vi "1_10_Racing_Main.vi"() -> ()   [LabVIEW 2024]
uses:
  <vilib>/vision/Measure.llb/Edge New.ctl
  <vilib>/vision/Measure.llb/Edge Options.ctl
  <vilib>/vision/Measure.llb/Edge Polarity.ctl
  <vilib>/Instr/_visa.llb/VISA Set IO Buffer Mask.ctl
  <vilib>/Instr/_visa.llb/VISA Flush IO Buffer Mask.ctl
  <vilib>/Platform/TimedLoop/XDataNode/timing_clust.ctl
  <vilib>/Platform/TimedLoop/XDataNode/nitl_modes.ctl
  <vilib>/Platform/TimedLoop/XDataNode/wakeup.ctl
  <vilib>/Analysis/geometry.llb/Point in Polygon (Array).vi
  <vilib>/Instr/_visa.llb/VISA Configure Serial Port (Instr).vi
  <vilib>/Utility/file.llb/Write Delimited Spreadsheet (string).vi
  <vilib>/Platform/TimedLoop/XDataNode/XDataNode.xnode
  <vilib>/Analysis/NI_AAL_Geometry.lvlib
  <vilib>/ptbypt/NI_PtbyPt.lvlib
  <vilib>/Platform/TimedLoop/XDataNode/XDNodeRunTimeDep.lvlib
panel:
  out "curve":bool
  out "3":bool
  out "1":bool
  out "2":bool
  in  "Tab Control":T1(tab)=enum."oCam"
  in  "RP2040_Com.":refnum<visa-resource-name>="COM1"
  in  "LiDAR_Com.":refnum<visa-resource-name>="COM7"
  in  "HLV_EStop":bool
  in  "HLV_AorM":bool=TRUE
  out "Alive_PCU":u8(slide)=187 scale=0.0..254.0
  out "PCU_GEAR":u8
  in  "HLV_GEAR":u8(slide) scale=0.0..2.0
  in  "HLV_SPEED(mps)":i16(slide)=180 scale=0.0..1000.0
  out "PCU_MODE":u8=1
  out "PCU_SPEED (mps)":dbl=0.41000000000000003
  out "PCU_STEER":i16=-1108
  in  "pure_Y":dbl=0.93
  in  "L":dbl=0.288
  in  "LAD":dbl=0.93
  out "PCU_EStop":bool
  out "PCU_ENC":i32=1739477
  out "pure_CMD(Deg)":dbl=-17.928890679668594
  out "steer(pwm)":i16=-1115
  out "LiDAR E-STOP":bool
  in  "pure_gain":dbl=1.0
  in  "stanley_Y":dbl=0.67
  in  "stanley_gain":dbl=1.0
  in  "stanley_speed":dbl=36.0
  in  "pure_min":dbl=0.38
  in  "steer_mean_size":i8=1
  out "stanley_CMD(Deg)":dbl=-0.8745447541552979
  out "Output_Spd_CMD(pwm)":dbl=163.8
  out "Near Point":dbl=-0.56975
  in  "stanley_con":dbl=0.023
  out "steer(deg)":i16(knob)=-16 scale=-25.0..25.0
  out "하위제어기 통신 패킷":string
  out "TX Data Cnt (byte)":u32=13
  out "RX Data Cnt (byte)":u32=17
  out "string":string
  in  "voxelsize":dbl=0.05
  out "Loop Time":u32=100
  out "Loop Time 2":u32=97
  out "LiDAR_ROI":cluster{"Array 2":dbl[], "Array":dbl[]}[](graph)=[{"Array 2"=[-650.0, -250.0, -250.0, -650.0, -650.0], "Array"=[-500.0, -500.0, 1000.0, 1000.0, -500.0]}, {"Array 2"=[], "Array"=[]}, {"Array 2"=[-200.0, 200.0, 200.0, -200.0, -200.0], "Array"=[280.0, 280.0, 1000.0, 1000.0, 280.0]}, {"Array 2"=[], "Array"=[]}, {"Array 2"=[250.0, 650.0, 650.0, 250.0, 250.0], "Array"=[-500.0, -500.0, 1000.0, 1000.0, -500.0]}, {"Array 2"=[], "Array"=[]}, {"Array 2"=[-200.0, 200.0, 200.0, -200.0, -200.0], "Array"=[80.0, 80.0, 280.0, 280.0, 80.0]}, {"Array 2"=[], "Array"=[]}]
  in  "euclid":dbl=200.0 format="%#_13g"
  in  "max_cluster_size":dbl=500.0 format="%#_13g"
  out "f_dis(m)":dbl[](array[numeric])
  out "right_edge_location":cluster{"X":sgl, "Y":sgl}[](array[cluster])=[{"X"=620.9575, "Y"=283.14465}, {"X"=620.9575, "Y"=283.14465}]
  out "left_edge_location":cluster{"X":sgl, "Y":sgl}[](array[cluster])
  out "mid_edge_location":cluster{"X":sgl, "Y":sgl}[](array[cluster])=[{"X"=95.05083, "Y"=287.6531}, {"X"=114.194305, "Y"=282.5482}]
  out "target center":dbl=105.0
  out "mid_line_edge":i32=105
  out "right_roi_dead":bool
  out "left_roi_dead":bool=TRUE
  out "right_line_edge":i32=621
  out "left_line_edge":i32
  out "mid_roi_dead":bool
  out "mid_far_edge":i32=634
  out "mid_near_edge":i32=539
  out "Image Out":T2(plugin-control)
  out "L_color":string="None"
  out "R_color":string="None"
  out "Right Edge Information":T3[](array[typedef])=[{"Location (Pixel)"={"X"=620.9575, "Y"=283.14465}, "Location (Real-World)"={"X"=620.9575, "Y"=283.14465}, "Distance (Pixel)"=38.249019622802734, "Distance (Real-World)"=38.249019622802734, "Strength"=27.666666666666668, "Noise"=12.666666666666666, "Rising?"=FALSE}, {"Location (Pixel)"={"X"=620.9575, "Y"=283.14465}, "Location (Real-World)"={"X"=620.9575, "Y"=283.14465}, "Distance (Pixel)"=38.249019622802734, "Distance (Real-World)"=38.249019622802734, "Strength"=27.666666666666668, "Noise"=9.0, "Rising?"=FALSE}] {"Distance (Real-World)" format="%.2f"; "Location (Real-World)"."Y" format="%.2g"; "Location (Real-World)"."X" format="%.2f"; "Noise" format="%.2f"; "Location (Pixel)"."Y" format="%.2g"; "Location (Pixel)"."X" format="%.2f"; "Strength" format="%.2f"; "Distance (Pixel)" format="%.2f"}
  out "Left Edge Information":T3[](array[typedef]) {"Distance (Real-World)" format="%.2f"; "Location (Real-World)"."Y" format="%.2g"; "Location (Real-World)"."X" format="%.2f"; "Noise" format="%.2f"; "Location (Pixel)"."Y" format="%.2g"; "Location (Pixel)"."X" format="%.2f"; "Strength" format="%.2f"; "Distance (Pixel)" format="%.2f"}
  out "Mid Edge Information":T3[](array[typedef])=[{"Location (Pixel)"={"X"=95.05083, "Y"=287.6531}, "Location (Real-World)"={"X"=95.05083, "Y"=287.6531}, "Distance (Pixel)"=20.751501083374023, "Distance (Real-World)"=20.751501083374023, "Strength"=56.666666666666664, "Noise"=6.0, "Rising?"=FALSE}, {"Location (Pixel)"={"X"=114.194305, "Y"=282.5482}, "Location (Real-World)"={"X"=114.194305, "Y"=282.5482}, "Distance (Pixel)"=40.56394577026367, "Distance (Real-World)"=40.56394577026367, "Strength"=41.666666666666664, "Noise"=5.666666507720947, "Rising?"=TRUE}] {"Distance (Real-World)" format="%.2f"; "Location (Real-World)"."Y" format="%.2g"; "Location (Real-World)"."X" format="%.2f"; "Noise" format="%.2f"; "Location (Pixel)"."Y" format="%.2g"; "Location (Pixel)"."X" format="%.2f"; "Strength" format="%.2f"; "Distance (Pixel)" format="%.2f"}
  out "left_able":bool
  out "right_able":bool
  out "left":bool
  out "rigt":bool
  out "kappa":dbl=0.009
  out "mid_far Edge Information":T3[](array[typedef]) {"Distance (Real-World)" format="%.2f"; "Location (Real-World)"."Y" format="%.2g"; "Location (Real-World)"."X" format="%.2f"; "Noise" format="%.2f"; "Location (Pixel)"."Y" format="%.2g"; "Location (Pixel)"."X" format="%.2f"; "Strength" format="%.2f"; "Distance (Pixel)" format="%.2f"}
  out "mid_near Edge Information":T3[](array[typedef]) {"Distance (Real-World)" format="%.2f"; "Location (Real-World)"."Y" format="%.2g"; "Location (Real-World)"."X" format="%.2f"; "Noise" format="%.2f"; "Location (Pixel)"."Y" format="%.2g"; "Location (Pixel)"."X" format="%.2f"; "Strength" format="%.2f"; "Distance (Pixel)" format="%.2f"}
  out "mid_near-edge_location":cluster{"X":sgl, "Y":sgl}[](array[cluster])
  out "mid_far-edge_location":cluster{"X":sgl, "Y":sgl}[](array[cluster])
  in  "right_line_center":i32=480
  in  "mid_line_center":i32=320
  in  "left_line_center":i32=160
  in  "Color Plane":i32(ring)=2 items=["Red", "Green", "Blue", "Hue", "Saturation", "Luminance", "Value", "Intensity"]
  in  "Right Descriptor":T4={"Global Rectangle"=[0, 0, 0, 0, 0], "Contours"=[{"ID"=enum."External", "Type"=2, "Coordinates"=[465, 285, 495, 285]}]} {"Contours"."Type" items=["No Selection", "Point", "Line", "Rectangle", "Oval", "Polygon", "Freehand Region", "Annulus", "Unused2", "Unused3", "Broken Line", "Freehand Line", "Rotated Rectangle"]}
  in  "Left Descriptor":T4={"Global Rectangle"=[0, 0, 0, 0], "Contours"=[{"ID"=enum."External", "Type"=2, "Coordinates"=[145, 285, 175, 285]}]} {"Contours"."Type" items=["No Selection", "Point", "Line", "Rectangle", "Oval", "Polygon", "Freehand Region", "Annulus", "Unused2", "Unused3", "Broken Line", "Freehand Line", "Rotated Rectangle"]}
  in  "Mid Descriptor":T4={"Global Rectangle"=[0, 0, 0, 0], "Contours"=[{"ID"=enum."External", "Type"=2, "Coordinates"=[305, 285, 335, 285]}]} {"Contours"."Type" items=["No Selection", "Point", "Line", "Rectangle", "Oval", "Polygon", "Freehand Region", "Annulus", "Unused2", "Unused3", "Broken Line", "Freehand Line", "Rotated Rectangle"]}
  in  "Lane Options":T5={"Edge Polarity"=0, "Kernel Size"=3, "Width"=3, "Minimum Edge Strength"=20.0, "Interpolation Type"=enum."Bilinear Fixed", "Data Processing Method"=enum."Average"} {"Edge Polarity" items=["All Edges", "Rising Edges", "Falling Edges"]; "Minimum Edge Strength" format="%.2f"; "Width" step=2; "Kernel Size" step=2}
  in  "Left Options":T5={"Edge Polarity"=0, "Kernel Size"=3, "Width"=3, "Minimum Edge Strength"=19.949999, "Interpolation Type"=enum."Bilinear Fixed", "Data Processing Method"=enum."Average"} {"Edge Polarity" items=["All Edges", "Rising Edges", "Falling Edges"]; "Minimum Edge Strength" format="%.2f"; "Width" step=2; "Kernel Size" step=2}
  in  "Right Options":T5={"Edge Polarity"=0, "Kernel Size"=3, "Width"=3, "Minimum Edge Strength"=20.0, "Interpolation Type"=enum."Bilinear Fixed", "Data Processing Method"=enum."Average"} {"Edge Polarity" items=["All Edges", "Rising Edges", "Falling Edges"]; "Minimum Edge Strength" format="%.2f"; "Width" step=2; "Kernel Size" step=2}
  in  "Left Process":T7(ring)=enum."Get First + Last Edge"
  in  "Lane Process":T7(ring)=enum."Get First + Last Edge"
  in  "Right Process":T7(ring)=enum."Get First + Last Edge"
  in  "Mid_near":T4={"Global Rectangle"=[0, 0, 0, 0], "Contours"=[{"ID"=enum."External", "Type"=2, "Coordinates"=[305, 360, 335, 360]}]} {"Contours"."Type" items=["No Selection", "Point", "Line", "Rectangle", "Oval", "Polygon", "Freehand Region", "Annulus", "Unused2", "Unused3", "Broken Line", "Freehand Line", "Rotated Rectangle"]}
  in  "Mid_far":T4={"Global Rectangle"=[0, 0, 0, 0], "Contours"=[{"ID"=enum."External", "Type"=2, "Coordinates"=[305, 320, 335, 320]}]} {"Contours"."Type" items=["No Selection", "Point", "Line", "Rectangle", "Oval", "Polygon", "Freehand Region", "Annulus", "Unused2", "Unused3", "Broken Line", "Freehand Line", "Rotated Rectangle"]}
  in  "mid_far Edge Options":T8={"Edge Polarity"=0, "Kernel Size"=3, "Width"=3, "Minimum Edge Strength"=10.0, "Interpolation Type"=enum."Bilinear Fixed", "Data Processing Method"=enum."Average"} {"Edge Polarity" items=["All Edges", "Rising Edges", "Falling Edges"]}
  in  "mid_near Edge Options":T8={"Edge Polarity"=0, "Kernel Size"=3, "Width"=3, "Minimum Edge Strength"=10.0, "Interpolation Type"=enum."Bilinear Fixed", "Data Processing Method"=enum."Average"} {"Edge Polarity" items=["All Edges", "Rising Edges", "Falling Edges"]}
  in  "배열":string[](array[string])=["INDEX", "Sys_Time", "SPD_CMD(pwm)", "PCU_SPD(mps)", "left_edge", "left_roi_dead", "mid_edge", "mid_roi_dead", "right_edge", "right_roi_dead", "PCU_MODE", "PCU_GEAR", "PCU_steer", "PCU_ENC", "steer(pwm)", "Alive_PCU", "PCU_Estop"]
  in  "LOG_Folder":path=path "C:/Users/LattePanda/Desktop/log"
  out "Size_init":i32=10
  in  "Data Save On/Off":bool
  in  "stop":bool=TRUE
  # "1/10 Autonomous Racing Program"
  # "※ 본 프로그램은 무료 배포 프로그램으로 상업용으로는 사용하지 말 것이며 사용 시 생기는 문제에 대해서 작성자는 책임지지 않습니다."
  # "HLV Control"
  # "Controller"
  # "Setting"
  # "2 : Auto Fail\n1 : Auto\n0 : Manual"
  # "0 : D 단\n1 : N 단\n2 : R 단"
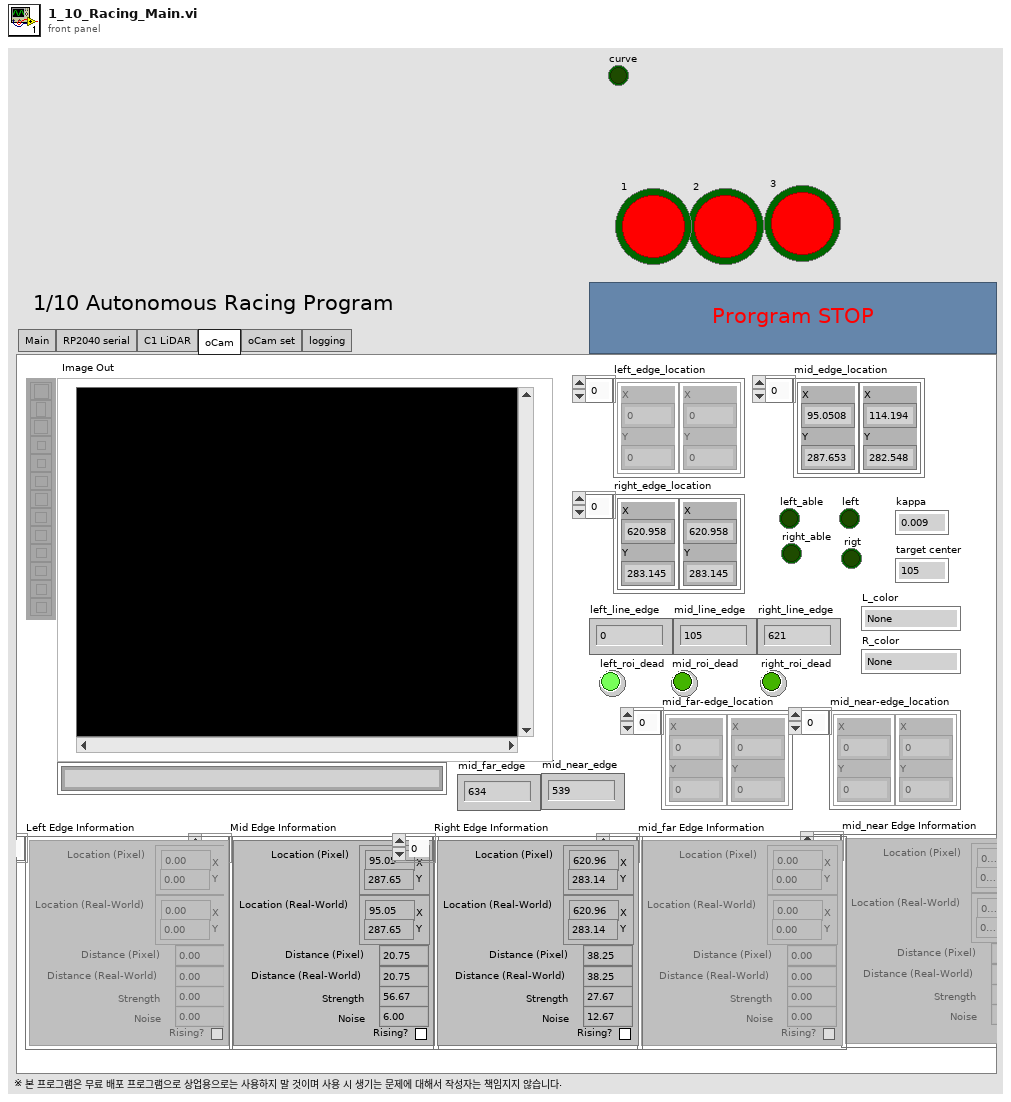
[diagram p1: front panel]
types:
  T1 = enum32{"Main", "RP2040 serial", "C1 LiDAR", "oCam", "oCam set", "logging"}
  T2 = typedef "IMAQ Image.ctl" = refnum<image>
  T3 = typedef "Edge New.ctl" = cluster{"Location (Pixel)":cluster{"X":sgl, "Y":sgl}, "Location (Real-World)":cluster{"X":sgl, "Y":sgl}, "Distance (Pixel)":dbl, "Distance (Real-World)":dbl, "Strength":dbl, "Noise":dbl, "Rising?":bool}
  T4 = typedef "ROI Descriptor" = cluster{"Global Rectangle":i32[], "Contours":cluster{"ID":enum32{"External", "Internal"}, "Type":u32, "Coordinates":i32[]}[]}
  T5 = typedef "Edge Options.ctl" = cluster{"Edge Polarity":T6, "Kernel Size":u32, "Width":u32, "Minimum Edge Strength":sgl, "Interpolation Type":enum32{"Zero Order", "Bilinear", "Quadratic", "Cubic", "Bilinear Fixed"}, "Data Processing Method":enum32{"Average", "Median"}}
  T6 = typedef "Edge Polarity.ctl" = u32
  T7 = enum16{"Get First Edge", "Get First + Last Edge", "Get All Edges", "Get Best Edge"}
  T8 = cluster{"Edge Polarity":u32, "Kernel Size":u32, "Width":u32, "Minimum Edge Strength":sgl, "Interpolation Type":enum32{"Zero Order", "Bilinear", "Quadratic", "Cubic", "Bilinear Fixed"}, "Data Processing Method":enum32{"Average", "Median"}}
  T9 = typedef "NI_AAL_Geometry.lvlib/Point in Polygon Position.ctl" = u16
  T10 = typedef "Image Type" = u32
  T11 = cluster{"Global Rectangle":i32[], cluster{"ID":enum32{"External", "Internal"}, "Type":u32, "Coordinates":i32[]}[]}
  T12 = cluster{"Global Rectangle":i32[], "배열":cluster{"ID":enum32{"External", "Internal"}, "Type":u32, "Coordinates":i32[]}[]}
  T13 = typedef "XDNodeRunTimeDep.lvlib/timing_clust.ctl" = cluster{"Expected End [f-1]":u64, "Actual End [f-1]":u64, "Finished Late? [f-1]":bool, "Expected End [i-1]":u64, "Actual End [i-1]":u64, "Finished Late? [i-1]":bool, "Expected Start [i]":u64, "Actual Start [i]":u64, "Expected Start [f]":u64, "Actual Start [f]":u64, "Source Name":string, "Structure Name":string, "Period":i64, "Deadline":i64, "Offset":i64, "Start":i64, "Priority":i32, "Timeout":i32, "Mode":T14, "Wakeup Reason":T15, "Error":errorcluster, "Source Type":string, "Secondary Source Type":string, "Global End Time":u64, "Global Start Time":u64, "Frame Duration":u64, "Iteration Duration":u64, "Assigned CPU":i32, "I/O Scan Engine Mode":u32}
  T14 = typedef "XDNodeRunTimeDep.lvlib/nitl_modes.ctl" = enum32{"No Change", "Process missed periods, maintain original phase", "Discard missed periods, maintain original phase", "Process missed periods, ignore original phase", "Discard missed periods, ignore original phase"}
  T15 = typedef "XDNodeRunTimeDep.lvlib/wakeup.ctl" = enum32{"Normal", "Aborted", "Asynchronous wakeup", "Timing source error", "Timed loop error", "Timeout"}
  T16 = cluster{"HLV_M/A_Status":u8, "HLV_EStop":u8, "HLV_Gear":u8, "HLV_Speed":i16, "HLV_Steer":i16, "HLV_Alive":u8}
  T17 = cluster{"ARD_M/A_Status":u8, "ARD_EStop":u8, "ARD_Gear":u8, "ARD_Speed":i16, "ARD_Steer":i16, "ARD_ENC":i32, "ARD_Alive":u8}
  T18 = typedef "VISA Flush IO Buffer Mask.ctl" = u16
  T19 = typedef "VISA Set IO Buffer Mask.ctl" = u16
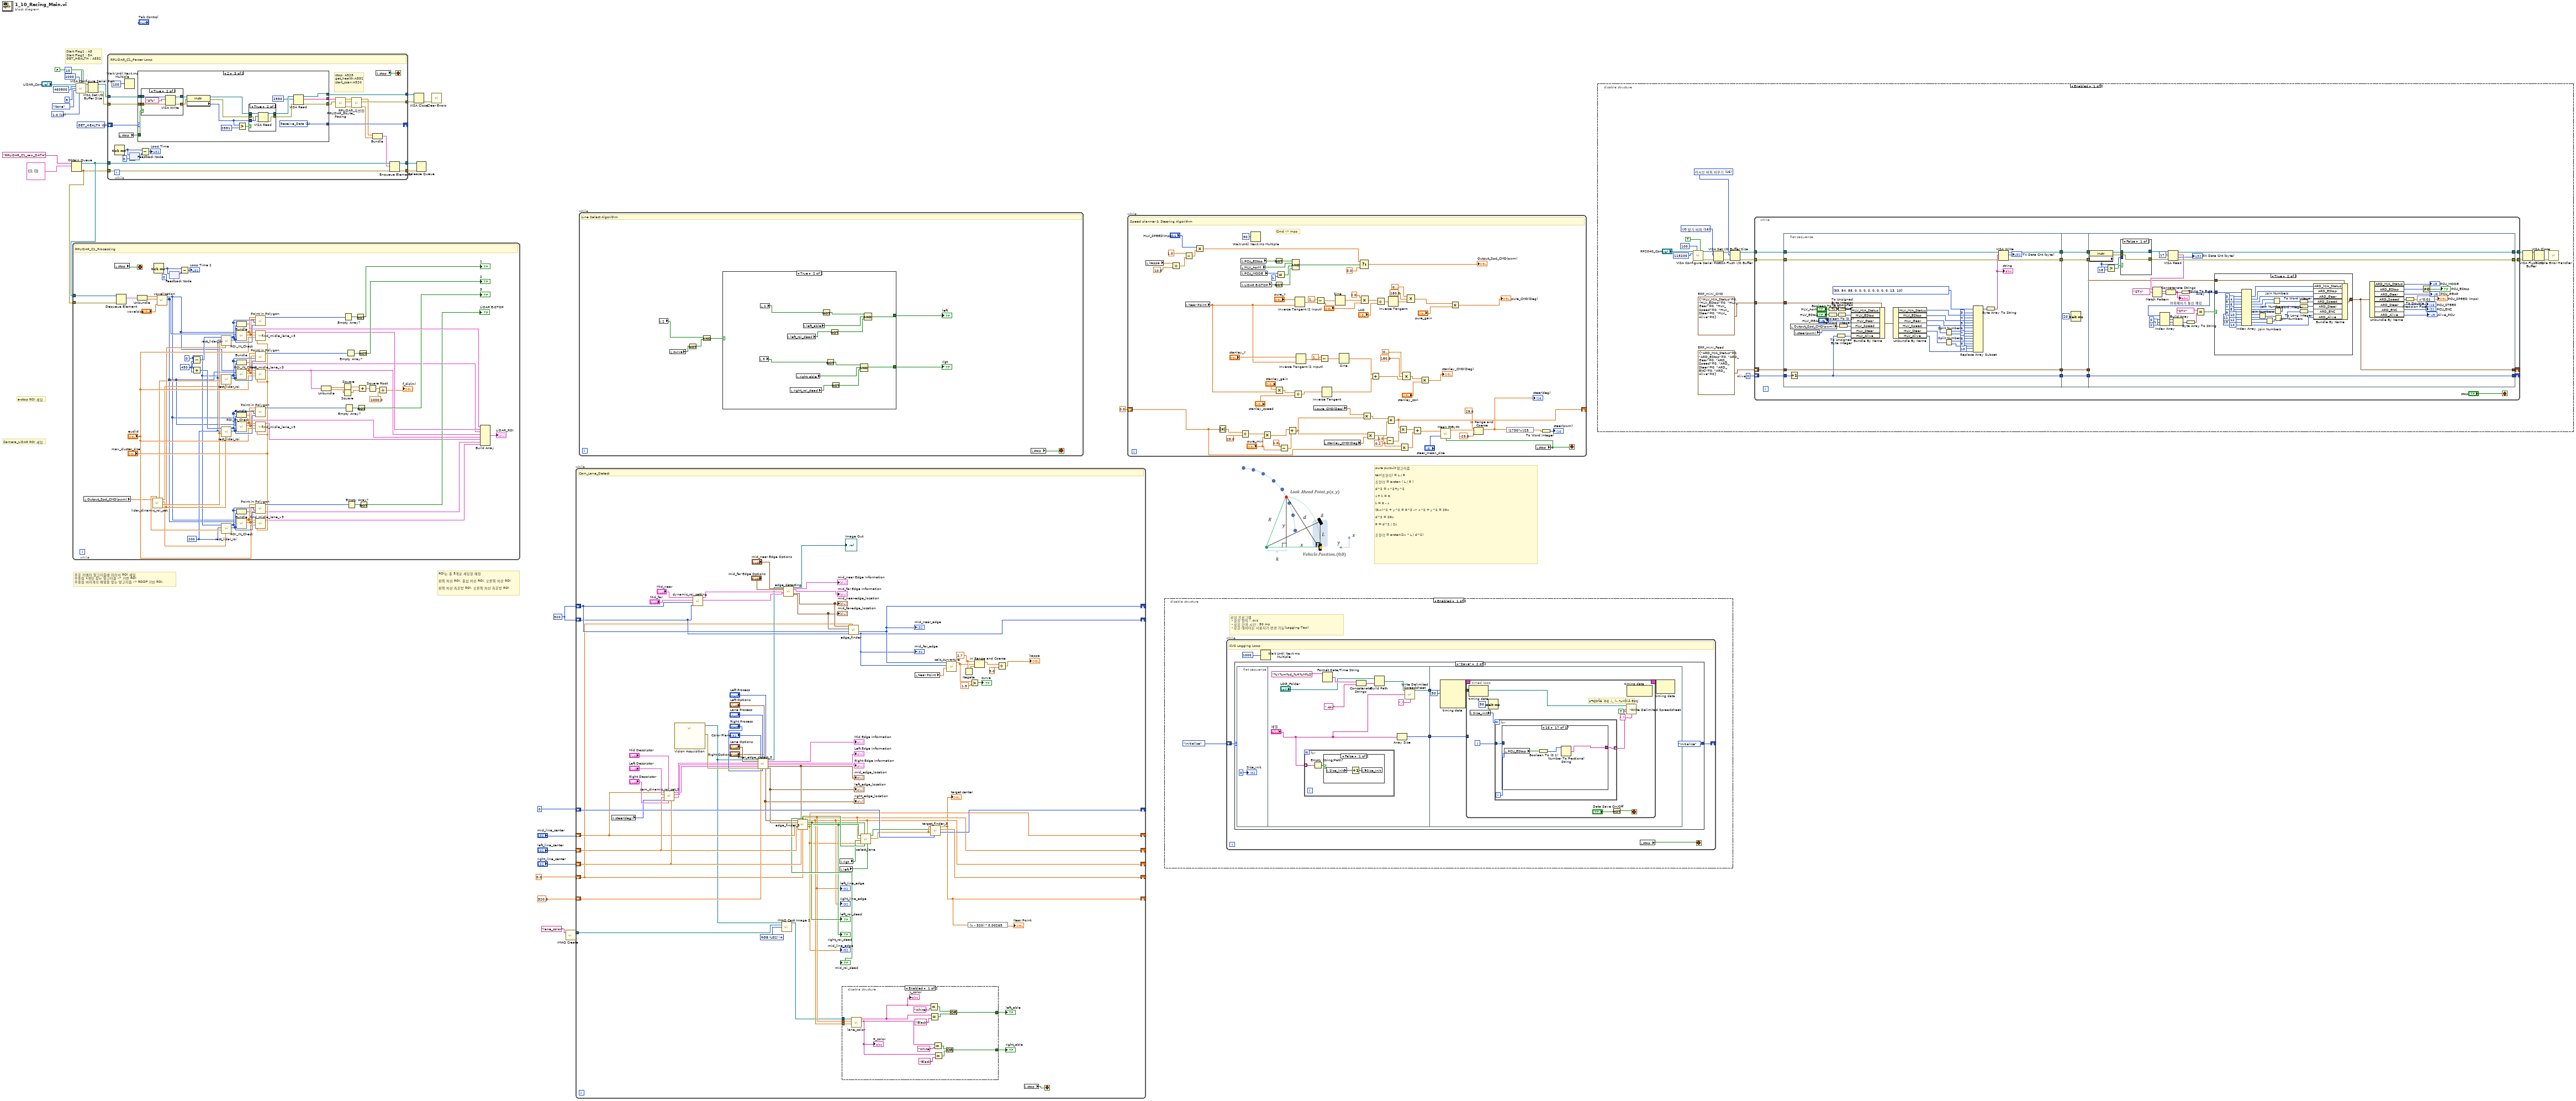
[diagram p0: block diagram]
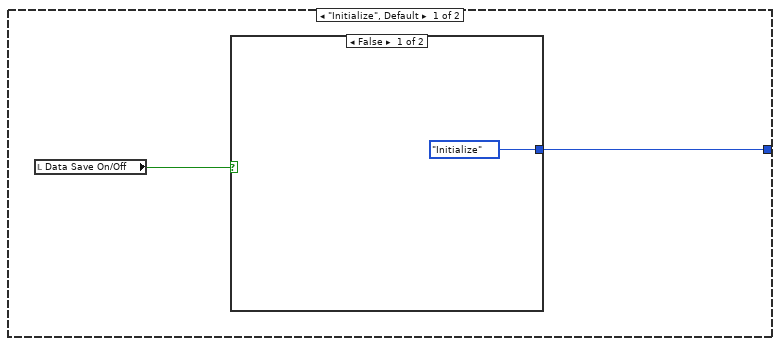
[diagram p2: hidden frame]
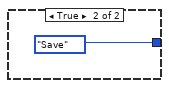
[diagram p3: hidden frame]
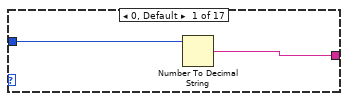
[diagram p5: hidden frame]
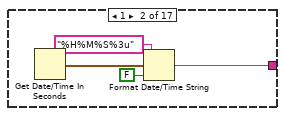
[diagram p6: hidden frame]
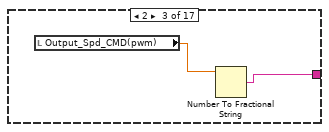
[diagram p7: hidden frame]
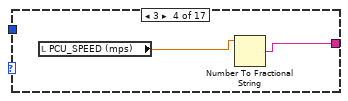
[diagram p8: hidden frame]
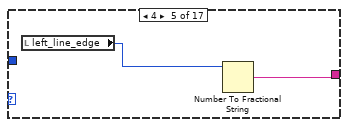
[diagram p9: hidden frame]
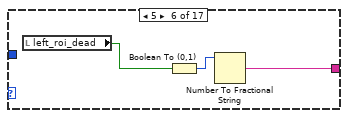
[diagram p10: hidden frame]
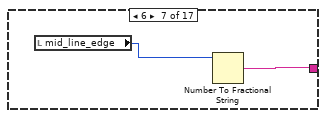
[diagram p11: hidden frame]
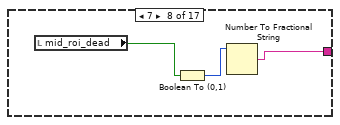
[diagram p12: hidden frame]
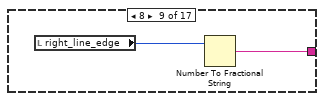
[diagram p13: hidden frame]
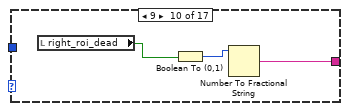
[diagram p14: hidden frame]
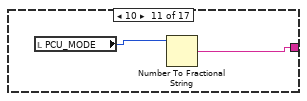
[diagram p15: hidden frame]
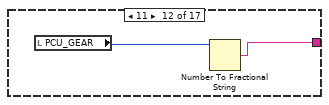
[diagram p16: hidden frame]
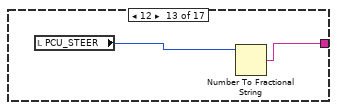
[diagram p17: hidden frame]
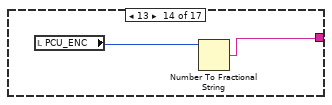
[diagram p18: hidden frame]
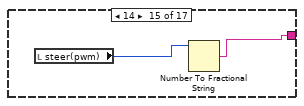
[diagram p19: hidden frame]
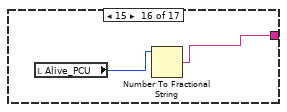
[diagram p20: hidden frame]
diagram:
  w2 = 320 ("left_line_center")
  w18 = u16 10 items=["1.0"=10, "1.5"=15, "2.0"=20] ("stop bits (10: 1 bit)")
  w20 = u16 0 items=["GET_HEALTH", "SCAN_START", "Receive_Data"]
  # "Camera_LiDAR ROI 세팅"
  # "e-stop ROI 세팅"
  # "ROI는 총 5개로 세팅할 예정\n\n왼쪽 차선 ROI, 중심 차선 ROI, 오른쪽 차선 ROI\n\n왼쪽 차선 측후방 ROI, 오른쪽 차선 측후방 ROI"
  # "추후 카메라 알고리즘에 따라서 ROI 세팅\n추종점 1개만 찾는 알고리즘 -> 가변 ROI\n추종점 여러개의 배열을 찾는 알고리즘 -> RDDF 기반 ROI."
  # "Start Flag1 : A5\nStart Flag2 : 5A \nGET_HEALTH : A552"
  # "pure pursuit 알고리즘\n\ntan(조향각) = L / R\n\n조향각 = arctan ( L / R )\n\nd^2 = x^2+y^2\n\nx+ k = R\n\nk = R - x\n\n(R-x)^2 + y^2 = R^2 -> x^2 + y^2 = 2Rx\n\nd^2 = 2Rx\n\nR = d^2 / 2x\n\n\n조향각 = arctan(2x * L / d^2)"
  n1 = Obtain Queue(name (unnamed)="RPLiDAR_C1_raw_DATA" ("이름(이름없음)"), element data type=cluster{dbl[], dbl[]} {[], []}) -> (queue out=w13:refnum<queue>, error out=w12:errorcluster)  [unwired: 3 in, 1 out]
  n2 = while {
    tunnel: w13 -> [w103]
    tunnel: w12 -> [w102]
    stop <- w101 stop-if-true
    w76 = u32 450 ("ms 배수")
    w51 = u32 0 ("ms 배수")
    w52 = u32 200 ("ms 배수")
    (unwired) u32 0 ("millisecond timer value")
    # "RPLIDAR_C1_Processing"
    n3 = local read "Output_Spd_CMD(pwm)"() -> (w47:dbl)
    n4 = local read "stop"() -> (w101:bool)
    n5 = Dequeue Element(queue=w103, error in (no error)=w102) -> (element=w97:cluster{dbl[], dbl[]})  [unwired: 1 in, 3 out]
    n6 = Unbundle(w97) -> (w96:dbl[], w95:dbl[])
    n7 = call "lidar_dinamic_roi_set.vi"("cmd"=w47) -> ("Z13_Half"=w57:dbl, "Z13_Ctr"=w58:dbl, "E_Half"=w53:dbl, "Z2_Half"=w55:dbl, "Z2_Ctr"=w56:dbl, "E_Ctr"=w54:dbl)  [unwired: 5 in]
    n8 = Tick Count (ms)() -> (millisecond timer value=w100:u32)
    n9 = call "voxelization.vi"("격자크기"="voxelsize", "Y"=w95, "X"=w96) -> ("voxeled_y"=w50:i32[], "voxeled_x"=w49:i32[])  [unwired: 7 in]
    n10 = feedback #1() -> (w99:u32)  [unwired: 1 in]
    n11 = feedback-in #1(w100) -> ()
    n12 = Subtract(x=w100, y=w99) -> (x-y=→"Loop Time 2":u32)
    n13 = Subtract(x=w51, y=w76) -> (x-y=w74:u32)
    n14 = Add(x=w51, y=w76) -> (x+y=w75:u32)
    n15 = call "rect_lidar_roi.vi"("y_range"=w57, "y_center"=w58, "x_range"=w52, "x_center"=w74) -> ("y"=w87:i32[], "x"=w88:i32[])  [unwired: 6 in]
    n16 = call "rect_lidar_roi.vi"("y_range"=w55, "y_center"=w56, "x_range"=w52, "x_center"=w51) -> ("y"=w89:i32[], "x"=w90:i32[])  [unwired: 6 in]
    n17 = call "rect_lidar_roi.vi"("y_range"=w57, "y_center"=w58, "x_range"=w52, "x_center"=w75) -> ("y"=w81:i32[], "x"=w80:i32[])  [unwired: 6 in]
    n18 = call "rect_lidar_roi.vi"("y_range"=w53, "y_center"=w54, "x_range"=w52, "x_center"=w51) -> ("y"=w66:i32[], "x"=w65:i32[])  [unwired: 6 in]
    n19 = Bundle("x"=w88, "y"=w87) -> (w83:cluster{"x":i32[], "y":i32[]})  [unwired: 1 in]
    n20 = call "ROI_IN_Check.vi"("도형Y좌표"=w87, "도형X좌표"=w88, "PCD_Y"=w50, "PCD_X"=w49) -> ("ROI_IN_Y"=w70:dbl[], "ROI_IN_X"=w71:dbl[])  [unwired: 5 in, 1 out]
    n21 = Bundle("x"=w90, "y"=w89) -> (w42:cluster{"x":i32[], "y":i32[]})  [unwired: 1 in]
    n22 = call "ROI_IN_Check.vi"("도형Y좌표"=w89, "도형X좌표"=w90, "PCD_Y"=w50, "PCD_X"=w49) -> ("ROI_IN_Y"=w72:dbl[], "ROI_IN_X"=w73:dbl[])  [unwired: 5 in, 1 out]
    n23 = Bundle("x"=w80, "y"=w81) -> (w46:cluster{"x":i32[], "y":i32[]})  [unwired: 1 in]
    n24 = call "ROI_IN_Check.vi"("도형Y좌표"=w81, "도형X좌표"=w80, "PCD_Y"=w50, "PCD_X"=w49) -> ("ROI_IN_Y"=w68:dbl[], "ROI_IN_X"=w69:dbl[])  [unwired: 5 in, 1 out]
    n25 = Bundle("x"=w65, "y"=w66) -> (w44:cluster{"x":i32[], "y":i32[]})  [unwired: 1 in]
    n26 = call "ROI_IN_Check.vi"("도형Y좌표"=w66, "도형X좌표"=w65, "PCD_Y"=w50, "PCD_X"=w49) -> ("ROI_IN_Y"=w60:dbl[], "ROI_IN_X"=w61:dbl[])  [unwired: 5 in, 1 out]
    n27 = call-poly <vilib>:"Point in Polygon.vi"("Polygon Y"=w87, "Polygon X"=w88, "Y"=w70, "X"=w71) -> ("Position"=w84:T9[])  [unwired: 6 in, 1 out]
    n28 = call "find_midle_lane_v3.vi"("max_cluster_size"="max_cluster_size", "euclid"="euclid", "LiDAR_Y"=w70, "LiDAR_X"=w71) -> ("filtered_data"=w67:cluster{dbl[], dbl[]})  [unwired: 2 in, 5 out]
    n29 = call-poly <vilib>:"Point in Polygon.vi"("Polygon Y"=w89, "Polygon X"=w90, "Y"=w72, "X"=w73) -> ("Position"=w93:T9[])  [unwired: 6 in, 1 out]
    n30 = call "find_midle_lane_v3.vi"("max_cluster_size"="max_cluster_size", "euclid"="euclid", "LiDAR_Y"=w72, "LiDAR_X"=w73) -> ("filtered_data"=w41:cluster{dbl[], dbl[]})  [unwired: 2 in, 5 out]
    n31 = call-poly <vilib>:"Point in Polygon.vi"("Polygon Y"=w81, "Polygon X"=w80, "Y"=w68, "X"=w69) -> ("Position"=w77:T9[])  [unwired: 6 in, 1 out]
    n32 = call "find_midle_lane_v3.vi"("max_cluster_size"="max_cluster_size", "euclid"="euclid", "LiDAR_Y"=w68, "LiDAR_X"=w69) -> ("filtered_data"=w45:cluster{dbl[], dbl[]})  [unwired: 2 in, 5 out]
    n33 = call-poly <vilib>:"Point in Polygon.vi"("Polygon Y"=w66, "Polygon X"=w65, "Y"=w60, "X"=w61) -> ("Position"=w64:T9[])  [unwired: 6 in, 1 out]
    n34 = call "find_midle_lane_v3.vi"("max_cluster_size"="max_cluster_size", "euclid"="euclid", "LiDAR_Y"=w60, "LiDAR_X"=w61) -> ("filtered_data"=w43:cluster{dbl[], dbl[]})  [unwired: 2 in, 5 out]
    n35 = Unbundle(w41) -> (w40:dbl[], w39:dbl[])
    n36 = Square(x=w40) -> (x^2=w38:dbl[])
    n37 = Square(x=w39) -> (x^2=w37:dbl[])
    n38 = Empty Array?(array=w84) -> (empty?=w85:bool)
    n39 = Empty Array?(array=w77) -> (empty?=w78:bool)
    n40 = Empty Array?(array=w93) -> (empty?=w92:bool)
    n41 = Empty Array?(array=w64) -> (empty?=w59:bool)
    n42 = Not(x=w85) -> (.not. x?=→"1":bool)
    n43 = Not(x=w78) -> (.not. x?=→"3":bool)
    n44 = Add(x=w38, y=w37) -> (x+y=w36:dbl[])
    n45 = Not(x=w92) -> (.not. x?=→"2":bool)
    n46 = Not(x=w59) -> (.not. x?=→"LiDAR E-STOP":bool)
    n47 = Square Root(x=w36) -> (sqrt(x)=w35:dbl[])
    n48 = Divide(x=w35, y=1000.0) -> (x/y=→"f_dis(m)":dbl[])
    n49 = Build Array(w83, w67, w42, w41, w46, w45, w44, w43) -> (→"LiDAR_ROI":cluster{"x":dbl[], "y":dbl[]}[])
  }
  n50 = call-poly "VISA Configure Serial Port"("VISA resource name"="LiDAR_Com.", "timeout (10sec)"=u32 1000, "termination char\n(0xA = '\\n' = LF)"=u8 10 ("termination char\n(0xA = '\\n' = LF)"), "Enable Termination\nChar (T)"=FALSE ("Enable Termination\nChar (T)"), "baud rate (9600)"=u32 460800, "data bits (8)"=u16 8, "parity (0:none)"=enum16{"None", "Odd", "Even", "Mark", "Space"}."None", "stop bits (10: 1 bit)"=w18) -> ("VISA resource name out"=w27:refnum<visa-resource-name>, "error out"=w26:errorcluster)  [unwired: 6 in]
  n51 = VISA Set I/O Buffer Size(VISA resource name=w27, error in (no error)=w26) -> (VISA resource name out=w22:refnum<visa-resource-name>, error out=w21:errorcluster)  [unwired: 2 in]
  n52 = while {
    tunnel: [w117] -> w31
    tunnel: [w116] -> w30
    tunnel: w22 -> [w125]
    tunnel: w21 -> [w124]
    shift-right: [w115] -> _
    shift-left: w20 -> [w126]
    tunnel: w13 -> [w108]
    tunnel: w12 -> [w107]
    tunnel: [w105] -> w15
    tunnel: [w104] -> w14
    stop <- w114 stop-if-true
    # "stop: A525\nget_health:A552\nstart_scan:A520"
    # "RPLIDAR_C1_Parser Loop"
    n53 = Tick Count (ms)() -> (millisecond timer value=w122:u32)
    n54 = local read "stop"() -> (w123:bool)
    n55 = Wait Until Next ms Multiple(millisecond multiple=u32 100 ("ms 배수")) -> ()  [unwired: 1 out]
    n56 = feedback #2(u32 0 ("millisecond timer value")) -> (w121:u32)
    n57 = feedback-in #2(w122) -> ()
    n58 = case shown="2" w126 {
      tunnel: w125 -> [w144 w162 w185]
      tunnel: w124 -> [w143 w161 w184]
      tunnel: [w145 w158 w171] -> w115
      tunnel: [w134 w159 w187] -> w116
      tunnel: [w133 w160 w186] -> w117
      tunnel: w123 -> [_ _ w183]
      tunnel: ["" ("read buffer") w156 w182] -> w113
      frame 0, Default {
        w127 = u16 0 items=["GET_HEALTH", "SCAN_START", "Receive_Data"]
        w128 = u16 1 items=["GET_HEALTH", "SCAN_START", "Receive_Data"]
        n59 = VISA Write(VISA resource name=w144, write buffer="¥R", error in (no error)=w143) -> (VISA resource name out=w138:refnum<visa-resource-name>, error out=w137:errorcluster)  [unwired: 1 out]
        n60 = flat-sequence {
          tunnel: w138 -> [w147]
          tunnel: w137 -> [w146]
          tunnel: [w147] -> w136
          tunnel: [w146] -> w135
          frame #0 {
            n61 = Wait (ms)(milliseconds to wait=u32 5 ("대기 시간 (ms)")) -> ()  [unwired: 1 out]
          }
        }
        n62 = property class="Instr"(reference=w136, error in=w135) -> (reference out=w141:refnum<visa-resource-name>, error out=w140:errorcluster, "Serial Settings:Number of Bytes at Serial Port"=w139:u32)
        n63 = VISA Read(VISA resource name=w141, byte count=w139, error in (no error)=w140) -> (VISA resource name out=w133:refnum<visa-resource-name>, read buffer=w130:string, error out=w134:errorcluster)  [unwired: 1 out]
        n64 = Equal?(x=w130, y="¥Z\u0003\u0000\u0000\u0000\u0006\u0000\u0000\u0000") -> (x = y?=w131:bool)
        n65 = Select(t=w128, s=w131, f=w127) -> (s? t:f=w145:u16)
      }
      frame 1 {
        w149 = u16 2 items=["GET_HEALTH", "SCAN_START", "Receive_Data"]
        w150 = u16 1 items=["GET_HEALTH", "SCAN_START", "Receive_Data"]
        w163 = "¥Z\u0005\u0000\u0000@"
        n66 = VISA Write(VISA resource name=w162, write buffer="¥ \u0000", error in (no error)=w161) -> (VISA resource name out=w165:refnum<visa-resource-name>, error out=w166:errorcluster)  [unwired: 1 out]
        n67 = flat-sequence {
          tunnel: w165 -> [w169]
          tunnel: w166 -> [w168]
          tunnel: [w169] -> w152
          tunnel: [w168] -> w151
          frame #0 {
            n68 = Wait (ms)(milliseconds to wait=u32 5 ("대기 시간 (ms)")) -> ()  [unwired: 1 out]
          }
        }
        n69 = property class="Instr"(reference=w152, error in=w151) -> (reference out=w155:refnum<visa-resource-name>, error out=w154:errorcluster, "Serial Settings:Number of Bytes at Serial Port"=w153:u32)
        n70 = VISA Read(VISA resource name=w155, byte count=w153, error in (no error)=w154) -> (VISA resource name out=w160:refnum<visa-resource-name>, read buffer=w156:string, error out=w159:errorcluster)  [unwired: 1 out]
        n71 = Match Pattern(string=w156, regular expression=w163) -> (match substring=w157:string)  [unwired: 1 in, 3 out]
        n72 = Equal?(x=w157, y=w163) -> (x = y?=w167:bool)
        n73 = Select(t=w149, s=w167, f=w150) -> (s? t:f=w158:u16)
      }
      frame 2 {
        w171 = u16 2 items=["GET_HEALTH", "SCAN_START", "Receive_Data"]
        n74 = case shown="True" w183 {
          tunnel: w185 -> [w196 w200]
          tunnel: w184 -> [w195 w199]
          tunnel: [w196 w198] -> w181
          tunnel: [w195 w197] -> w180
          frame False {
          }
          frame True {
            n75 = VISA Write(VISA resource name=w200, write buffer="¥%", error in (no error)=w199) -> (VISA resource name out=w198:refnum<visa-resource-name>, error out=w197:errorcluster)  [unwired: 1 out]
          }
        }
        n76 = property class="Instr"(reference=w181, error in=w180) -> (reference out=w176:refnum<visa-resource-name>, error out=w175:errorcluster, "Serial Settings:Number of Bytes at Serial Port"=w177:u32)
        n77 = Greater?(x=w177, y=u32 2551) -> (0:w179:bool)
        n78 = case shown="True" w179 {
          tunnel: w176 -> [w189 w194]
          tunnel: w177 -> [_ w193]
          tunnel: w175 -> [w188 w192]
          tunnel: [w189 w191] -> w174
          tunnel: [w188 w190] -> w173
          frame False {
          }
          frame True {
            n79 = VISA Read(VISA resource name=w194, byte count=w193, error in (no error)=w192) -> (VISA resource name out=w191:refnum<visa-resource-name>, error out=w190:errorcluster)  [unwired: 2 out]
          }
        }
        n80 = VISA Read(VISA resource name=w174, byte count=u32 2550, error in (no error)=w173) -> (VISA resource name out=w186:refnum<visa-resource-name>, read buffer=w182:string, error out=w187:errorcluster)  [unwired: 1 out]
      }
    }
    n81 = Subtract(x=w122, y=w121) -> (x-y=→"Loop Time":u32)
    n82 = call "PRLIDAR_5byte_Pasing.vi"("RPLIDAR_Data"=w113) -> ("Distance(mm)"=w111:dbl[], "Theta(deg)"=w112:dbl[])  [unwired: 9 in]
    n83 = call "RPLiDAR_축변환.vi"("Distance(mm)"=w111, "Theta(deg)"=w112) -> ("Y"=w109:dbl[], "X"=w110:dbl[])  [unwired: 8 in]
    n84 = Bundle("X"=w110, "Y"=w109) -> (w106:cluster{"X":dbl[], "Y":dbl[]})  [unwired: 1 in]
    n85 = local read "stop"() -> (w114:bool)
    n86 = Enqueue Element(queue=w108, element=w106, error in (no error)=w107) -> (queue out=w105:refnum<queue>, error out=w104:errorcluster)  [unwired: 1 in, 1 out]
  }
  n87 = VISA Close(VISA resource name=w31, error in (no error)=w30) -> (error out=w32:errorcluster)
  n88 = Release Queue(queue=w15, error in (no error)=w14) -> ()  [unwired: 1 in, 3 out]
  n89 = call <vilib>:"Clear Errors.vi"("error in (no error)"=w32) -> ()  [unwired: 5 in, 2 out]
  n90 = call "IMAQ Create"("Image Name"="lane_color") -> ("New Image"=w3:T2)  [unwired: 4 in, 1 out]
  n91 = while {
    shift-right: [w231] -> _
    shift-left: "mid_line_center" -> [w253]
    shift-right: [w239] -> _
    shift-left: "left_line_center" -> [w255]
    shift-right: [w238] -> _
    shift-left: "right_line_center" -> [w258]
    shift-right: [w257] -> _
    shift-left: 0.0 ("roi_reset") -> [w214]
    shift-right: [w254] -> _
    shift-left: 0 -> [w256]
    shift-right: [w211] -> _
    shift-left: 320.0 ("Lane_center 2") -> [w252]
    tunnel: w3 -> [w234]
    shift-right: [w213] -> _
    shift-left: w2 -> [w219]
    shift-right: [w212] -> _
    shift-left: w2 -> [w218]
    stop <- w248 stop-if-true
    w208 = 2.7 ("upper limit")
    w233 = T10 4 items=["Grayscale (U8)", "Grayscale (I16)", "Grayscale (SGL)", "Complex (CSG)", "RGB (U32)", "HSL (U32)", "RGB (U64)", "Grayscale (U16)"] ("Image Type")
    # "Cam_Lane_Detect"
    n92 = local read "steer(deg)"() -> (w229:i16)
    n93 = call "cam_dinamic_roi_set_3.vi"("Right_center"=w258, "Right Descriptor"="Right Descriptor", "Lane Descriptor"="Mid Descriptor", "steer(deg)"=w229, "Left_center"=w255, "Left Descriptor"="Left Descriptor", "Lane_center"=w253) -> ("Right"=w262:T11, "Left"=w264:T11, "Mid"=w235:T11)  [unwired: 2 in]
    n94 = call "Vision Acquisition"() -> ("Image Out"=w230:T2, "error out"=w273:errorcluster)  [unwired: 25 in, 1 out]
    n95 = call "dynamic_roi_setting.vi"("right_line_center"=w218, "left_line_center"=w219, "mid_far Descriptor"="Mid_far", "mid_near Descriptor"="Mid_near") -> ("far_roi"=w224:T12, "near_roi"=w225:T12)  [unwired: 6 in]
    n96 = call "filter_edge_detect_3.vi"("image in"=w230, "mid Lane Options"="Lane Options", "right Lane Descriptor"=w262, "left Lane Descriptor"=w264, "mid Lane Descriptor"=w235, "error in (no error)"=w273, "Color Plane"="Color Plane", "Lane_center"=w252, "Lane Process"="Lane Process", "Right Process"="Right Process", "Left Options"="Left Options", "Right Options"="Right Options", "Left Process"="Left Process") -> ("right_edge_location"=w241:cluster{"X":sgl, "Y":sgl}[], "image out"=w216:T2, "Mid Edge Information"=→"Mid Edge Information":T3[], "Left Edge Information"=→"Left Edge Information":T3[], "Right Edge Information"=→"Right Edge Information":T3[], "mid_edge_location"=w243:cluster{"X":sgl, "Y":sgl}[], "left_edge_location"=w242:cluster{"X":sgl, "Y":sgl}[])
    "mid_edge_location" <- w243
    "left_edge_location" <- w242
    "right_edge_location" <- w241
    n97 = call "IMAQ Cast Image 2"("Image Src"=w230, "Image Dst"=w234, "Image Type"=w233) -> ("Image Dst Out"=w232:T2)  [unwired: 11 in, 1 out]
    n98 = call "edge_detecting.vi"("Image In"=w216, "mid_near Edge Options"="mid_near Edge Options", "mid_far Edge Options"="mid_far Edge Options", "mid_near Descriptor"=w225, "mid_far Descriptor"=w224) -> ("Image Out"=→"Image Out":T2, "mid_near Edge Information"=→"mid_near Edge Information":T3[], "mid_far Edge Information"=→"mid_far Edge Information":T3[], "mid_near-edge_location"=w221:cluster{"X":sgl, "Y":sgl}[], "mid_far-edge_location"=w220:cluster{"X":sgl, "Y":sgl}[])  [unwired: 17 in, 1 out]
    "mid_near-edge_location" <- w221
    "mid_far-edge_location" <- w220
    n99 = call "edge_finder_3.vi"("right_edge_location"=w241, "mid_edge_location"=w243, "left_edge_location"=w242, "Mid_center in"=w253, "Left_center in"=w255, "Right_center in"=w258, "Reset_ROI"=w214) -> ("mid_roi_dead"=w251:bool, "left_line_center"=w239:dbl, "right_line_center"=w238:dbl, "left_roi_dead"=w250:bool, "right_roi_dead"=w249:bool, "mid_center out"=w231:dbl)  [unwired: 2 in, 1 out]
    "mid_roi_dead" <- w251
    "left_line_edge" <- w239
    "right_line_edge" <- w238
    "left_roi_dead" <- w250
    "right_roi_dead" <- w249
    "mid_line_edge" <- w231
    n100 = local read "rigt"() -> (w244:bool)
    n101 = local read "left"() -> (w245:bool)
    n102 = disable-structure shown="Enabled" {
      disable-tunnel: w232 -> [w289 _]
      disable-tunnel: w239 -> [w288 _]
      disable-tunnel: w238 -> [w287 _]
      disable-tunnel: [w276 w290] -> w237
      disable-tunnel: [w275 w290] -> w236
      frame Enabled {
        n103 = call "lane_color.vi"("Rx"=w287, "Lx"=w288, "image in"=w289) -> ("R_color"=w279:string, "L_color"=w284:string)  [unwired: 7 in]
        "L_color" <- w284
        "R_color" <- w279
        n104 = Equal?(x=w284, y="White") -> (x = y?=w283:bool)
        n105 = Equal?(x=w284, y="Black") -> (x = y?=w282:bool)
        n106 = Equal?(x=w279, y="White") -> (x = y?=w278:bool)
        n107 = Equal?(x=w279, y="Black") -> (x = y?=w277:bool)
        n108 = Or(x=w278, y=w277) -> (x .or. y?=w275:bool)
        n109 = Or(x=w283, y=w282) -> (x .or. y?=w276:bool)
      }
      frame Disabled {
        w290 = TRUE
      }
    }
    "left_able" <- w237
    "right_able" <- w236
    n110 = call "edge_finder.vi"("roi_reset"=w214, "pre_mid_far_edge"=w218, "pre_mid_near_edge"=w219, "current_mid_far_location"=w220, "current_mid_near_location"=w221) -> ("mid_far_edge"=w212:i32, "mid_near_edge"=w213:i32)  [unwired: 3 in, 2 out]
    "mid_near_edge" <- w213
    "mid_far_edge" <- w212
    n111 = call "select_lane.vi"("left"=w245, "right_line_edge"=w238, "mid_roi_dead"=w251, "left_roi_dead"=w250, "mid_center in"=w231, "rigt"=w244, "left_line_edge"=w239, "right_roi_dead"=w249) -> ("target_center"=w247:dbl, "roi_reset"=w246:bool)  [unwired: 2 in]
    n112 = local read "Near Point"() -> (w210:dbl)
    n113 = call "target_finder_3.vi"("prev_count"=w256, "Lane_center"=w247, "roi_dead"=w246, "Lane_center in"=w247) -> ("next_count"=w254:i32, "Reset_ROI"=w257:dbl, "Lane_center out"=w211:dbl)  [unwired: 5 in]
    "target center" <- w211
    n114 = call "calc_curvarture.vi"("Near Point"=w210, "mid_far_edge"=w212, "mid_near_edge"=w213) -> ("kappa"=w204:dbl)  [unwired: 8 in]
    n115 = Negate(x=w208) -> (-x=w209:dbl)
    n116 = expression code="(x - 320) * 0.00265"(w211) -> (→"Near Point":dbl)
    n117 = Greater?(x=w204, y=1.5) -> (0:→"curve":bool)
    n118 = In Range and Coerce(upper limit=w208, x=w204, lower limit=w209) -> (coerced(x)=w205:dbl)  [unwired: 1 out]
    n119 = Divide(x=w205, y=3.0) -> (x/y=→"kappa":dbl)
    n120 = local read "stop"() -> (w248:bool)
  }
  n121 = while "While 루프" {
    stop <- w297 stop-if-true
    # "Line Select Algorithm"
    n122 = local read "2"() -> (w294:bool)
    n123 = local read "curve"() -> (w293:bool)
    n124 = Not(x=w293) -> (.not. x?=w292:bool)
    n125 = And(x=w294, y=w292) -> (x .and. y?=w291:bool)
    n126 = case shown="True" w291 {
      tunnel: [w298 w308] -> w296
      tunnel: [w298 w299] -> w295
      frame False {
        w298 = FALSE
      }
      frame True {
        n127 = local read "3"() -> (w309:bool)
        n128 = local read "1"() -> (w310:bool)
        n129 = local read "left_roi_dead"() -> (w305:bool)
        n130 = local read "right_roi_dead"() -> (w301:bool)
        n131 = local read "right_able"() -> (w302:bool)
        n132 = local read "left_able"() -> (w306:bool)
        n133 = Not(x=w310) -> (.not. x?=w307:bool)
        n134 = Not(x=w309) -> (.not. x?=w303:bool)
        n135 = Not(x=w305) -> (.not. x?=w304:bool)
        n136 = Not(x=w301) -> (.not. x?=w300:bool)
        n137 = Compound Arithmetic op=AND(w303, w302, w300) -> (w299:bool)
        n138 = Compound Arithmetic op=AND(w307, w306, w304) -> (w308:bool)
      }
    }
    "left" <- w296
    "rigt" <- w295
    n139 = local read "stop"() -> (w297:bool)
  }
  n140 = while {
    shift-right: [w333] -> _
    shift-left: 0.0 -> [w330]
    stop <- w328 stop-if-true
    w331 = 0.2 ("y")
    # "Cmd -> mps"
    # "Speed planner & Steering Algorithm"
    n141 = local read "kappa"() -> (w315:dbl)
    n142 = Divide(x=w315, y=10.0 ("x")) -> (x/y=w313:dbl)
    n143 = Subtract(x=1.0, y=w313) -> (x-y=w312:dbl)
    n144 = local read "Near Point"() -> (w357:dbl)
    n145 = Multiply(x="HLV_SPEED(mps)", y=w312) -> (x*y=w311:dbl)
    n146 = Absolute Value(x=w330) -> (abs(x)=w344:dbl)
    n147 = Divide(x=w344, y=25.0) -> (x/y=w343:dbl)
    n148 = local read "PCU_EStop"() -> (w385:bool)
    n149 = local read "HLV_AorM"() -> (w388:bool)
    n150 = local read "PCU_MODE"() -> (w369:u8)
    n151 = local read "LiDAR E-STOP"() -> (w383:bool)
    n152 = Wait Until Next ms Multiple(millisecond multiple=u32 50 ("ms 배수")) -> ()  [unwired: 1 out]
    n153 = Multiply(x=w343, y="pure_min") -> (x*y=w342:dbl)
    n154 = Not(x=w385) -> (.not. x?=w386:bool)
    n155 = Not(x=w383) -> (.not. x?=w384:bool)
    n156 = Multiply(x="stanley_gain", y=w357) -> (x*y=w356:dbl)
    n157 = Equal?(x=w369, y=u8 1) -> (x = y?=w366:bool)
    n158 = Subtract(x=1.0, y="pure_min") -> (x-y=w339:dbl)
    n159 = Add(x=w342, y=w339) -> (x+y=w337:dbl)
    n160 = Compound Arithmetic op=AND ("복합 연산")(w386, w388, w366, w384) -> (w387:bool)
    n161 = Divide(x=w356, y="stanley_speed") -> (x/y=w354:dbl)
    n162 = Inverse Tangent (2 Input)(1:w357, 2:"pure_Y") -> (0:w375:dbl)
    n163 = Inverse Tangent (2 Input)(1:w357, 2:"stanley_Y") -> (0:w359:dbl)
    n164 = local read "pure_CMD(Deg)"() -> (w336:dbl)
    n165 = Subtract(x=1.5707963267948966, y=w375) -> (x-y=w370:dbl)
    n166 = Subtract(x=1.5707963267948966, y=w359) -> (x-y=w360:dbl)
    n167 = Inverse Tangent(1:w354) -> (0:w352:dbl)
    n168 = local read "stanley_CMD(Deg)"() -> (w338:dbl)
    n169 = Sine(x=w370) -> (sin(x)=w372:dbl)
    n170 = Sine(x=w360) -> (sin(x)=w353:dbl)
    n171 = Select(t=w311, s=w387, f=0.0) -> (s? t:f=→"Output_Spd_CMD(pwm)":dbl)
    n172 = Compound Arithmetic op=MULTIPLY(2.0, w372, "L") -> (w371:dbl)
    n173 = Multiply(x=w336, y=w337) -> (x*y=w347:dbl)
    n174 = Multiply(x=w337, y=w338) -> (x*y=w346:dbl)
    n175 = Add(x=w353, y=w352) -> (x+y=w349:dbl)
    n176 = Divide(x=w371, y="LAD") -> (x/y=w376:dbl)
    n177 = Subtract(x=1.0, y=w331) -> (x-y=w334:dbl)
    n178 = Add(x=w347, y=w346) -> (x+y=w333:dbl)
    n179 = Inverse Tangent(1:w376) -> (0:w377:dbl)
    n180 = Multiply(x=w333, y=w334) -> (x*y=w332:dbl)
    n181 = Multiply(x=w331, y=w330) -> (x*y=w329:dbl)
    n182 = Compound Arithmetic op=MULTIPLY(0.3183098861837907, 180.0, w349) -> (w322:dbl)
    n183 = Compound Arithmetic op=MULTIPLY(0.3183098861837907, 180.0, w377) -> (w364:dbl)
    n184 = Add(x=w332, y=w329) -> (x+y=w319:dbl)
    n185 = Multiply(x=w322, y="stanley_con") -> (x*y=→"stanley_CMD(Deg)":dbl)
    n186 = Multiply(x=w364, y="pure_gain") -> (x*y=→"pure_CMD(Deg)":dbl)
    n187 = local read "stop"() -> (w328:bool)
    n188 = call <vilib>:"Mean PtByPt.vi"("x"=w319, "sample length"="steer_mean_size", "initialize"=w328) -> ("mean"=w325:dbl)  [unwired: 1 in, 1 out]
    n189 = In Range and Coerce(upper limit=25.0, x=w325, lower limit=-25.0) -> (coerced(x)=w318:dbl)  [unwired: 1 out]
    "steer(deg)" <- w318
    n190 = expression code="(1730*x)/25"(w318) -> (w348:dbl)
    n191 = To Word Integer(number=w348) -> (16bit integer=→"steer(pwm)":i16)
  }
  n192 = disable-structure shown="Enabled" {
    frame Enabled {
      # "로깅 프로그램\n - 로깅 형식 : .cvs\n - 로깅 간격 시간 : 50 ms\n - 로깅 데이터는 사용자가 변경 가능(Logging Tap)"
      n193 = while {
        shift-right: [w393] -> _
        shift-left: enum16{"Initialize", "Save"}."Initialize" -> [w394]
        stop <- w392 stop-if-true
        # "CVS Logging Loop"
        n194 = case shown="\"Save\"" w394 {
          tunnel: [w396 enum16{"Initialize", "Save"}."Initialize"] -> w393
          frame "Initialize", Default {
            n195 = local read "Data Save On/Off"() -> (w397:bool)
            n196 = case shown="False" w397 {
              tunnel: [enum16{"Initialize", "Save"}."Initialize" enum16{"Initialize", "Save"}."Save"] -> w396
              frame False {
              }
              frame True {
              }
            }
          }
          frame "Save" {
            n197 = flat-sequence {
              tunnel: [w412] -> w402
              tunnel: [w411] -> w401
              tunnel: w402 -> [w422]
              tunnel: w401 -> [w421]
              frame #0 {
                "Size_init" <- 0 ("Size_init")
              }
              frame #1 {
                n198 = for {
                  tunnel: "배열" -> [w415] mode=indexing
                  n199 = Empty String/Path?(string/path=w415) -> (empty?=w414:bool)
                  n200 = case shown="False" w414 {
                    frame False {
                      n201 = local read "Size_init"() -> (w417:i32)
                      n202 = Increment(x=w417) -> (x+1=w416:i32)
                      n203 = local write "Size_init"(w416) -> ()
                    }
                    frame True {
                    }
                  }
                }
                n204 = Format Date/Time String(time format string (%c)="%Y%m%d_%H%M%S" ("시간 포맷 문자열 (%c)")) -> (date/time string=w408:string)  [unwired: 2 in]
                n205 = Concatenate Strings(w408, ".csv" ("string")) -> (w407:string)
                n206 = Build Path(base path="LOG_Folder", name or relative path=w407) -> (appended path=w409:path)
                n207 = Array Size(array="배열") -> (size(s)=w411:i32)
                n208 = call-poly <vilib>:"Write Delimited Spreadsheet.vi"("file path (dialog if empty)"=w409, "1D data"="배열", "delimiter (\\t)"="," ("delimiter (\\t)")) -> ("new file path (Not A Path if cancelled)"=w412:path)  [unwired: 11 in, 1 out]
              }
              frame #2 {
                n209 = node-c288(i64 50 ("Period")) -> (w420:T13)  [unwired: 3 in]
                n210 = timed-loop {
                  tunnel: w422 -> [w431]
                  tunnel: w421 -> [_]
                  timing: w420 -> [_]
                  timing-out: [_] -> w419
                  i -> [w429]
                  stop <- w424 stop-if-true
                  # "p³tÇ0Ñä´DÇ ,\\¸ l­„½XÕìÅ È¥Ç"
                  n211 = node-c288() -> ()  [unwired: 1 in, 1 out]
                  n212 = local read "Size_init"() -> (w426:i32)
                  n213 = Wait (ms)(milliseconds to wait=u32 50) -> ()  [unwired: 1 out]
                  n214 = for {
                    N: w426 -> [_]
                    tunnel: w429 -> [w435]
                    tunnel: [w434] -> w428 mode=indexing
                    i -> [w436]
                    n215 = case shown="16" w436 {
                      tunnel: w435 -> [w438 _ _ _ _ _ _ _ _ _ _ _ _ _ _ _ _]
                      tunnel: [w437 w439 w444 w446 w448 w450 w453 w456 w458 w461 w463 w465 w467 w469 w471 w473 w476] -> w434
                      frame 0, Default {
                        n216 = Number To Decimal String(number=w438) -> (decimal integer string=w437:string)  [unwired: 1 in]
                      }
                      frame 1 {
                        n217 = Get Date/Time In Seconds() -> (seconds since 1Jan1904=w441:timestamp)
                        n218 = Format Date/Time String(time format string (%c)="%H%M%S%3u", seconds (now)=w441, UTC format=FALSE) -> (date/time string=w439:string)
                      }
                      frame 2 {
                        n219 = local read "Output_Spd_CMD(pwm)"() -> (w443:dbl)
                        n220 = Number To Fractional String(number=w443) -> (F-format string=w444:string)  [unwired: 3 in]
                      }
                      frame 3 {
                        n221 = local read "PCU_SPEED (mps)"() -> (w445:dbl)
                        n222 = Number To Fractional String(number=w445) -> (F-format string=w446:string)  [unwired: 3 in]
                      }
                      frame 4 {
                        n223 = local read "left_line_edge"() -> (w447:i32)
                        n224 = Number To Fractional String(number=w447) -> (F-format string=w448:string)  [unwired: 3 in]
                      }
                      frame 5 {
                        n225 = local read "left_roi_dead"() -> (w449:bool)
                        n226 = Boolean To (0,1)(Boolean=w449) -> (0, 1=w451:i16)
                        n227 = Number To Fractional String(number=w451) -> (F-format string=w450:string)  [unwired: 3 in]
                      }
                      frame 6 {
                        n228 = local read "mid_line_edge"() -> (w452:i32)
                        n229 = Number To Fractional String(number=w452) -> (F-format string=w453:string)  [unwired: 3 in]
                      }
                      frame 7 {
                        n230 = local read "mid_roi_dead"() -> (w454:bool)
                        n231 = Boolean To (0,1)(Boolean=w454) -> (0, 1=w455:i16)
                        n232 = Number To Fractional String(number=w455) -> (F-format string=w456:string)  [unwired: 3 in]
                      }
                      frame 8 {
                        n233 = local read "right_line_edge"() -> (w457:i32)
                        n234 = Number To Fractional String(number=w457) -> (F-format string=w458:string)  [unwired: 3 in]
                      }
                      frame 9 {
                        n235 = local read "right_roi_dead"() -> (w459:bool)
                        n236 = Boolean To (0,1)(Boolean=w459) -> (0, 1=w460:i16)
                        n237 = Number To Fractional String(number=w460) -> (F-format string=w461:string)  [unwired: 3 in]
                      }
                      frame 10 {
                        n238 = local read "PCU_MODE"() -> (w462:u8)
                        n239 = Number To Fractional String(number=w462) -> (F-format string=w463:string)  [unwired: 3 in]
                      }
                      frame 11 {
                        n240 = local read "PCU_GEAR"() -> (w464:u8)
                        n241 = Number To Fractional String(number=w464) -> (F-format string=w465:string)  [unwired: 3 in]
                      }
                      frame 12 {
                        n242 = local read "PCU_STEER"() -> (w466:i16)
                        n243 = Number To Fractional String(number=w466) -> (F-format string=w467:string)  [unwired: 3 in]
                      }
                      frame 13 {
                        n244 = local read "PCU_ENC"() -> (w468:i32)
                        n245 = Number To Fractional String(number=w468) -> (F-format string=w469:string)  [unwired: 3 in]
                      }
                      frame 14 {
                        n246 = local read "steer(pwm)"() -> (w470:i16)
                        n247 = Number To Fractional String(number=w470) -> (F-format string=w471:string)  [unwired: 3 in]
                      }
                      frame 15 {
                        n248 = local read "Alive_PCU"() -> (w472:u8)
                        n249 = Number To Fractional String(number=w472) -> (F-format string=w473:string)  [unwired: 3 in]
                      }
                      frame 16 {
                        n250 = local read "PCU_EStop"() -> (w475:bool)
                        n251 = Boolean To (0,1)(Boolean=w475) -> (0, 1=w474:i16)
                        n252 = Number To Fractional String(number=w474) -> (F-format string=w476:string)  [unwired: 3 in]
                      }
                    }
                  }
                  n253 = Not(x="Data Save On/Off") -> (.not. x?=w424:bool)
                  n254 = call-poly <vilib>:"Write Delimited Spreadsheet.vi"("file path (dialog if empty)"=w431, "1D data"=w428, "append to file? (new file:F)"=TRUE, "delimiter (\\t)"="," ("delimiter (\\t)")) -> ()  [unwired: 10 in, 2 out]
                  n255 = node-c288() -> ()  [unwired: 1 in, 1 out]
                }
                n256 = node-c288(w419) -> ()  [unwired: 1 out]
              }
            }
          }
        }
        n257 = Wait Until Next ms Multiple(millisecond multiple=u32 1000) -> ()  [unwired: 1 out]
        n258 = local read "stop"() -> (w392:bool)
      }
    }
    frame Disabled {
    }
  }
  n259 = disable-structure shown="Enabled" {
    frame Enabled {
      w493 = T16 {"HLV_M/A_Status"=0, "HLV_EStop"=0, "HLV_Gear"=0, "HLV_Speed"=0, "HLV_Steer"=0, "HLV_Alive"=0}  # ERP_mini_CMD
      w494 = T17 {"ARD_M/A_Status"=0, "ARD_EStop"=0, "ARD_Gear"=0, "ARD_Speed"=0, "ARD_Steer"=0, "ARD_ENC"=0, "ARD_Alive"=0}  # ERP_mini_Feed
      w481 = u8 0  # Alive
      w484 = T18 16 items=["리시브 버퍼 비우기"=16, "전달 버퍼 디바이스에 쓰기"=32, "리시브 버퍼 비우기(I/O 없음)"=64, "전달 버퍼 비우기"=128] ("Mask")
      w487 = T19 16 items=["I/O 받기 버퍼"=16, "I/O 전달 버퍼"=32, "I/O 받기와 전달 버퍼"=48] ("Mask")
      n260 = call-poly "VISA Configure Serial Port"("VISA resource name"="RP2040_Com.", "timeout (10sec)"=u32 100, "Enable Termination\nChar (T)"=TRUE ("Enable Termination\nChar (T)"), "baud rate (9600)"=u32 115200) -> ("VISA resource name out"=w489:refnum<visa-resource-name>, "error out"=w488:errorcluster)  [unwired: 10 in]
      n261 = VISA Set I/O Buffer Size(VISA resource name=w489, mask (16)=w487, error in (no error)=w488) -> (VISA resource name out=w486:refnum<visa-resource-name>, error out=w485:errorcluster)  [unwired: 1 in]
      n262 = VISA Flush I/O Buffer(VISA resource name=w486, mask (16)=w484, error in (no error)=w485) -> (VISA resource name out=w498:refnum<visa-resource-name>, error out=w482:errorcluster)
      n263 = while {
        tunnel: w498 -> [w518]
        tunnel: w482 -> [w517]
        tunnel: [w512] -> w497
        tunnel: [w511] -> w496
        shift-right: [w507] -> _
        shift-left: w494 -> [w509]
        tunnel: w493 -> [w506]
        shift-right: [w502] -> _
        shift-left: w481 -> [w505]
        stop <- "stop" stop-if-true
        n264 = flat-sequence {
          tunnel: [w547] -> w515
          tunnel: [w546] -> w513
          tunnel: w518 -> [w549]
          tunnel: w517 -> [w548]
          tunnel: [w544] -> w510
          tunnel: w509 -> [w544]
          tunnel: w506 -> [w543]
          tunnel: w505 -> [w541]
          tunnel: [w540] -> w503
          tunnel: [w565] -> w516
          tunnel: w515 -> [w565]
          tunnel: [w564] -> w514
          tunnel: w513 -> [w564]
          tunnel: w510 -> [w563]
          tunnel: [w563] -> w508
          tunnel: [w562] -> w504
          tunnel: w503 -> [w562]
          tunnel: w516 -> [w585]
          tunnel: w514 -> [w584]
          tunnel: [w607] -> w512
          tunnel: [w606] -> w511
          tunnel: w508 -> [w587]
          tunnel: [w586] -> w507
          tunnel: [w576] -> w502
          tunnel: w504 -> [w576]
          frame #0 {
            n265 = Increment(x=w541) -> (x+1=w540:u8)
            n266 = local read "Output_Spd_CMD(pwm)"() -> (w519:dbl)
            n267 = local read "steer(pwm)"() -> (w521:i16)
            n268 = Boolean To (0,1)(Boolean="HLV_AorM") -> (0, 1=w542:i16)
            n269 = Boolean To (0,1)(Boolean="HLV_EStop") -> (0, 1=w533:i16)
            n270 = To Unsigned Byte Integer(number=w540) -> (unsigned 8bit integer=w555:u8)
            n271 = To Unsigned Byte Integer(number=w542) -> (unsigned 8bit integer=w534:u8)
            n272 = To Unsigned Byte Integer(number=w533) -> (unsigned 8bit integer=w531:u8)
            n273 = To Word Integer(number=w519) -> (16bit integer=w520:i16)
            n274 = Bundle By Name(cluster=w543, "HLV_M/A_Status"=w534, "HLV_EStop"=w531, "HLV_Gear"="HLV_GEAR", "HLV_Speed"=w520, "HLV_Steer"=w521, "HLV_Alive"=w555) -> (w550:T16)
            n275 = Unbundle By Name(w550) -> ("HLV_M/A_Status"=w530:u8, "HLV_EStop"=w529:u8, "HLV_Gear"=w528:u8, "HLV_Speed"=w536:i16, "HLV_Steer"=w535:i16, "HLV_Alive"=w522:u8)
            n276 = Split Number(x=w536) -> (hi(x)=w527:u8, lo(x)=w526:u8)
            n277 = Split Number(x=w535) -> (hi(x)=w525:u8, lo(x)=w524:u8)
            n278 = Replace Array Subset(array=u8[] [83, 84, 88, 0, 0, 0, 0, 0, 0, 0, 0, 13, 10] ("unsigned byte array"), new element #1=w530, index #1=3, new element #2=w529, index #2=4, new element #3=w528, index #3=5, new element #4=w527, index #4=6, new element #5=w526, index #5=7, new element #6=w525, index #6=8, new element #7=w524, index #7=9, new element #8=w522, index #8=10) -> (w558:u8[])
            n279 = Byte Array To String(unsigned byte array=w558) -> (string=w559:string)
            "string" <- w559
            n280 = VISA Write(VISA resource name=w549, write buffer=w559, error in (no error)=w548) -> (VISA resource name out=w547:refnum<visa-resource-name>, return count=→"TX Data Cnt (byte)":u32, error out=w546:errorcluster)
          }
          frame #1 {
            n281 = Wait (ms)(milliseconds to wait=u32 20 ("대기 시간 (ms)")) -> ()  [unwired: 1 out]
          }
          frame #2 {
            n282 = property class="Instr"(reference=w585, error in=w584) -> (reference out=w583:refnum<visa-resource-name>, error out=w582:errorcluster, "Serial Settings:Number of Bytes at Serial Port"=w577:u32)
            n283 = Greater?(x=w577, y=u32 18) -> (0:w579:bool)
            n284 = case shown="False" w579 {
              tunnel: w583 -> [w609 w614]
              tunnel: w582 -> [w608 w613]
              tunnel: [w609 w612] -> w581
              tunnel: [w608 w611] -> w580
              tunnel: w577 -> [_ w610]
              frame False {
              }
              frame True {
                n285 = VISA Read(VISA resource name=w614, byte count=w610, error in (no error)=w613) -> (VISA resource name out=w612:refnum<visa-resource-name>, error out=w611:errorcluster)  [unwired: 2 out]
              }
            }
            n286 = VISA Read(VISA resource name=w581, byte count=u32 17, error in (no error)=w580) -> (VISA resource name out=w607:refnum<visa-resource-name>, read buffer=w605:string, return count=→"RX Data Cnt (byte)":u32, error out=w606:errorcluster)
            n287 = Match Pattern(string=w605, regular expression="STX") -> (match substring=w602:string, after substring=w603:string)  [unwired: 1 in, 2 out]
            n288 = Concatenate Strings(w602, w603) -> (w601:string)
            "하위제어기 통신 패킷" <- w601
            n289 = String To Byte Array(string=w601) -> (unsigned byte array=w589:u8[])
            n290 = Index Array(array=w589, index #1=0, index #2=1, index #3=2) -> (element #1=w595:u8, element #2=w594:u8, element #3=w593:u8)
            n291 = Build Array(w595, w594, w593) -> (w592:u8[])
            n292 = Byte Array To String(unsigned byte array=w592) -> (string=w590:string)
            n293 = Equal?(x="STX", y=w590) -> (x = y?=w588:bool)
            n294 = case shown="True" w588 {
              tunnel: w589 -> [_ w650]
              tunnel: [w615 w649] -> w586
              tunnel: w587 -> [w615 w648]
              frame False {
              }
              frame True {
                n295 = Index Array(array=w650, index #1=3, index #2=4, index #3=5, index #4=6, index #5=7, index #6=8, index #7=9, index #8=10, index #9=11, index #10=12, index #11=13, index #12=14) -> (element #1=w637:u8, element #2=w636:u8, element #3=w635:u8, element #4=w634:u8, element #5=w633:u8, element #6=w631:u8, element #7=w630:u8, element #8=w622:u8, element #9=w621:u8, element #10=w620:u8, element #11=w619:u8, element #12=w624:u8)
                n296 = Join Numbers(hi=w622, lo=w621) -> ((hi.lo)=w618:u16)
                n297 = Join Numbers(hi=w620, lo=w619) -> ((hi.lo)=w617:u16)
                n298 = Join Numbers(hi=w634, lo=w633) -> ((hi.lo)=w632:u16)
                n299 = Join Numbers(hi=w631, lo=w630) -> ((hi.lo)=w629:u16)
                n300 = Join Numbers(hi=w618, lo=w617) -> ((hi.lo)=w616:u32)
                n301 = To Word Integer(number=w632) -> (16bit integer=w641:i16)
                n302 = To Word Integer(number=w629) -> (16bit integer=w640:i16)
                n303 = To Long Integer(number=w616) -> (32bit integer=w623:i32)
                n304 = Bundle By Name(cluster=w648, "ARD_M/A_Status"=w637, "ARD_EStop"=w636, "ARD_Gear"=w635, "ARD_Speed"=w641, "ARD_Steer"=w640, "ARD_ENC"=w623, "ARD_Alive"=w624) -> (w649:T17)
              }
            }
            n305 = Unbundle By Name(w586) -> ("ARD_M/A_Status"=→"PCU_MODE":u8, "ARD_EStop"=w569:u8, "ARD_Gear"=→"PCU_GEAR":u8, "ARD_Speed"=w573:i16, "ARD_Steer"=→"PCU_STEER":i16, "ARD_ENC"=→"PCU_ENC":i32, "ARD_Alive"=→"Alive_PCU":u8)
            n306 = To Double Precision Float(number=w573) -> (double precision float=w574:dbl)
            n307 = expression code="x*0.01"(w574) -> (→"PCU_SPEED (mps)":dbl)
            n308 = Not Equal To 0?(x=w569) -> (x != 0?=→"PCU_EStop":bool)
          }
        }
      }
      n309 = VISA Flush I/O Buffer(VISA resource name=w497, error in (no error)=w496) -> (VISA resource name out=w499:refnum<visa-resource-name>, error out=w500:errorcluster)  [unwired: 1 in]
      n310 = VISA Close(VISA resource name=w499, error in (no error)=w500) -> (error out=w495:errorcluster)
      n311 = call <vilib>:"Simple Error Handler.vi"("error in (no error)"=w495) -> ()  [unwired: 4 in, 5 out]
    }
    frame Disabled {
    }
  }
